vi "Logic for Default Case - Multiple Converter.vi"(11 "error in":errorcluster) -> (15 "error out":errorcluster)   [LabVIEW 2021, in "Converter.lvlib"]
uses:
  Converter.lvlib
  <vilib>/Utility/traverseref.llb/TRef TravTarget.ctl
  <vilib>/Utility/traverseref.llb/VI Scripting - Traverse.lvlib
  Converter Reusables/Converter Reusables.lvlib
  Path Functions/Path Functions.lvlib
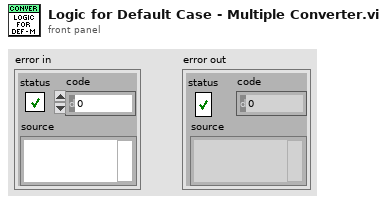
[diagram p1: front panel]
types:
  T1 = typedef "TRef TravTarget.ctl" = enum16{"FP", "BD", "Other"}
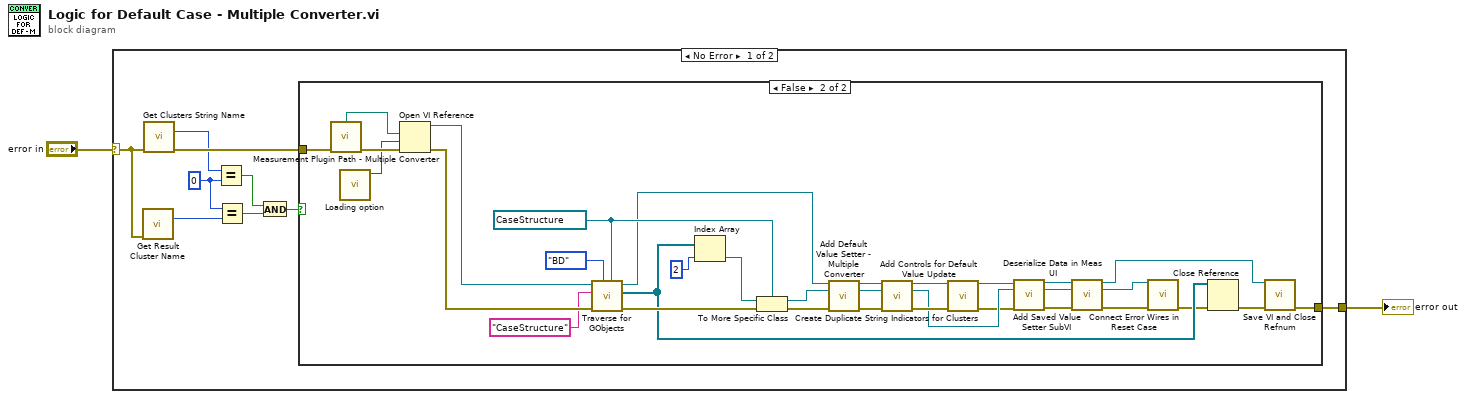
[diagram p0: block diagram]
diagram:
  n1 = case shown="No Error" "error in" {
    selector: "error in" -> [w10 w46]
    tunnel: [w11 w46] -> w2
    frame No Error {
      w4 = 0 ("y")
      n2 = call "Get Result Cluster Name.vi"("error in"=w10) -> ("array size"=w7:i32)  [unwired: 12 in, 2 out]
      n3 = call "Get Clusters String Name.vi"("error in"=w10) -> ("array size"=w8:i32, "error out"=w9:errorcluster)  [unwired: 12 in, 1 out]
      n4 = Equal?(x=w8, y=w4) -> (x = y?=w6:bool)
      n5 = Equal?(x=w4, y=w7) -> (x = y?=w3:bool)
      n6 = And(x=w6, y=w3) -> (x .and. y?=w5:bool)
      n7 = case shown="False" w5 {
        tunnel: [w12 w40] -> w11
        tunnel: w9 -> [w12 w22]
        frame True {
        }
        frame False {
          w42 = refnum<vi> refnum ("Other Refnum")
          n8 = call "Measurement Plugin Path - Multiple Converter.vi"("error in"=w22) -> ("measurement ui"=w24:path, "error out"=w23:errorcluster)  [unwired: 2 in, 11 out]
          n9 = call "Loading option.vi"() -> ("options"=w13:i32)  [unwired: 11 in]
          n10 = Open VI Reference(vi path=w24, options=w13, error in (no error)=w23) -> (vi reference=w36:refnum<vi>, error out=w45:errorcluster)  [unwired: 3 in]
          n11 = call <vilib>:"Traverse for GObjects.vi"("Other Refnum"=w42, "Traverse Target"=TRef_TravTarget."BD", "error in (no error)"=w45, "Class Name"="CaseStructure", "VI Refnum"=w36) -> ("error out"=w41:errorcluster, "References"=w30:refnum<vi>[], "dup VI Refnum"=w21:refnum<vi>)  [unwired: 3 in, 1 out]
          n12 = Index Array(array=w30, index=2) -> (element=w38:refnum<vi>)
          n13 = To More Specific Class(target class=w42, reference=w38, error in=w41) -> (specific class reference=w20:refnum<vi>, error out=w19:errorcluster)
          n14 = call "Add Default Value Setter - Multiple Converter.vi"("vi in"=w21, "case sel refnum in"=w20, "error in"=w19) -> ("vi out"=w17:refnum<vi>, "case sel refnum out"=w16:refnum<vi>, "error out"=w18:errorcluster)  [unwired: 10 in]
          n15 = call "Add Controls for Default Value Update.vi"("vi refnum in"=w17, "case sel refnum in"=w16, "error in"=w18) -> ("vi refnum out"=w35:refnum<vi>, "case sel refnum out"=w33:refnum<vi>, "error out"=w37:errorcluster)  [unwired: 10 in]
          n16 = call "Create Duplicate String Indicators for Clusters.vi"("ui vi ref in"=w35, "error in"=w37) -> ("ui vi ref out"=w34:refnum<vi>, "error out"=w27:errorcluster)  [unwired: 12 in]
          n17 = call "Add Saved Value Setter SubVI.vi"("vi in"=w34, "case sel refnum in"=w33, "error in"=w27) -> ("vi out"=w32:refnum<vi>, "case sel refnum out"=w31:refnum<vi>, "error out"=w28:errorcluster)  [unwired: 10 in]
          n18 = call "Deserialize Data in Meas UI.vi"("vi refnum in"=w32, "case sel refnum in"=w31, "error in"=w28) -> ("vi refnum out"=w14:refnum<vi>, "case sel refnum out"=w15:refnum<vi>, "error out"=w25:errorcluster)  [unwired: 10 in]
          n19 = call "Connect Error Wires in Reset Case.vi"("case sel refnum in"=w15, "error in"=w25) -> ("error out"=w26:errorcluster)  [unwired: 12 in, 1 out]
          n20 = Close Reference(reference=w30, error in (no error)=w26) -> (error out=w29:errorcluster)
          n21 = call "Save VI and Close Refnum.vi"("vi refnum"=w14, "error in"=w29) -> ("error out"=w40:errorcluster)  [unwired: 13 in]
        }
      }
    }
    frame Error {
    }
  }
  "error out" <- w2
